vi "demo 1.vi"() -> ()   [LabVIEW 2026, in "My Singleton Module.lvlib"]
uses:
  My Singleton Module.lvlib
panel:
  out "Status":string
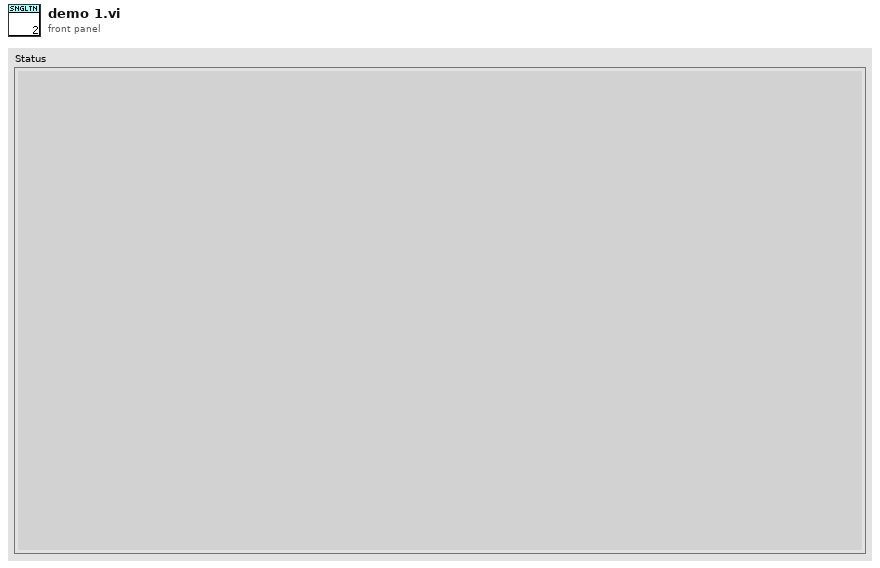
[diagram p1: front panel]
types:
  T1 = typedef "My Singleton Module.lvlib/Broadcast Events--cluster.ctl" = cluster{"Module Did Init":refnum<user-event>, "Status Updated":refnum<user-event>, "Error Reported":refnum<user-event>, "Did Something":refnum<user-event>, "Module Did Stop":refnum<user-event>, "Update Module Execution Status":refnum<user-event>}
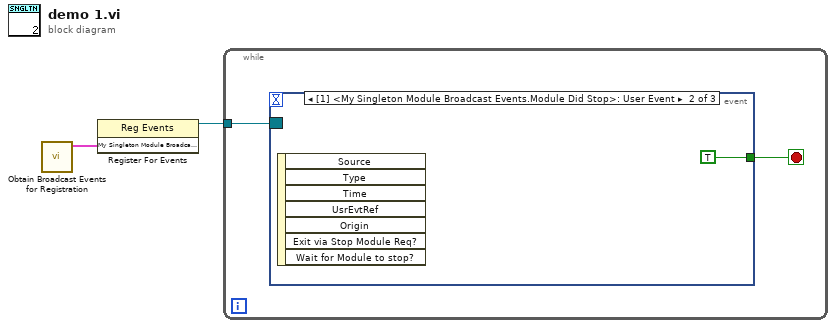
[diagram p0: block diagram]
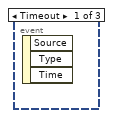
[diagram p2: hidden frame]
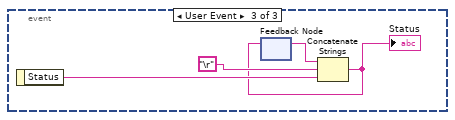
[diagram p3: hidden frame]
diagram:
  n1 = call "Obtain Broadcast Events for Registration.vi"() -> ("My Singleton Module Broadcast Events"=w2:T1)  [unwired: 9 in, 2 out]
  n2 = register-events(w2) -> (reference out=w1:refnum<event-registration>)  [unwired: 2 in, 1 out]
  n3 = while {
    tunnel: w1 -> [w4]
    stop <- w3 stop-if-true
    n4 = event shown="[1] <My Singleton Module Broadcast Events.Module Did Stop>: User Event" {
      selector: w4 -> [_ _ _]
      dyn-events: _ -> [_ _ _]
      timeout: _ -> [_ _ _]
      tunnel: [_ TRUE _] -> w3
      event Timeout {
        n5 = event-data() -> ()  [unwired: 1 in, 3 out]
      }
      event User Event {
        n6 = event-data() -> ()  [unwired: 1 in, 7 out]
      }
      event User Event {
        n7 = event-data() -> ("Status"=w9:string)  [unwired: 1 in]
        n8 = feedback #1() -> (w8:string)  [unwired: 1 in]
        n9 = Concatenate Strings(w8, "\r", w9) -> (w6:string)
        "Status" <- w6
        n10 = feedback-in #1(w6) -> ()
      }
    }
  }
